vi "SimpleReadWrite.vi"() -> ()   [LabVIEW 2015]
panel:
  out "读取缓冲区":string
  in  "读取的字节数":u32=1024
  in  "指令":string="*IDN?"
  in  "VISA资源名称":refnum<visa-resource-name>
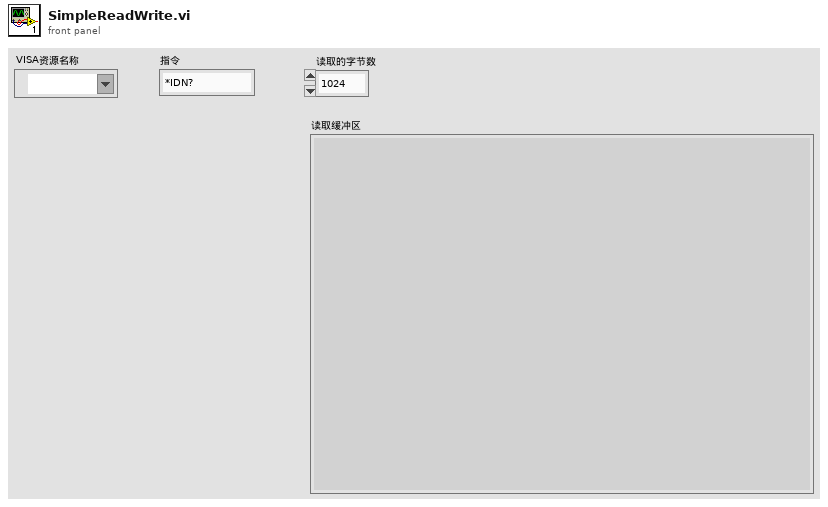
[diagram p1: front panel]
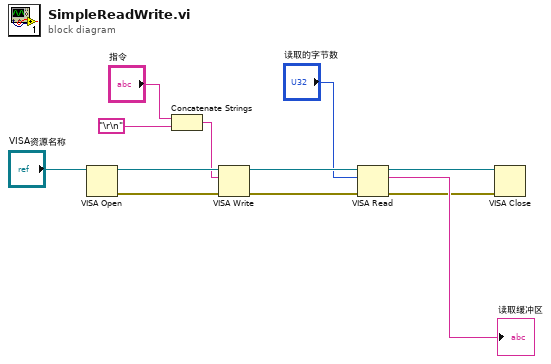
[diagram p0: block diagram]
diagram:
  n1 = VISA Open(VISA resource name="VISA资源名称") -> (VISA resource name=w11:refnum<visa-resource-name>, error out=w3:errorcluster)  [unwired: 4 in]
  n2 = Concatenate Strings("指令", "\r\n") -> (w4:string)
  n3 = VISA Write(VISA resource name=w11, write buffer=w4, error in (no error)=w3) -> (VISA resource name out=w10:refnum<visa-resource-name>, error out=w2:errorcluster)  [unwired: 1 out]
  n4 = VISA Read(VISA resource name=w10, byte count="读取的字节数", error in (no error)=w2) -> (VISA resource name out=w9:refnum<visa-resource-name>, read buffer=→"读取缓冲区":string, error out=w1:errorcluster)  [unwired: 1 out]
  n5 = VISA Close(VISA resource name=w9, error in (no error)=w1) -> ()  [unwired: 1 out]
